vi "TestGit01.vi"() -> ()   [LabVIEW 2025]
uses:
  <vilib>/Analysis/NI_AALPro.lvlib
panel:
  in  "stop":bool
  out "Waveform Chart":dbl[](graph)
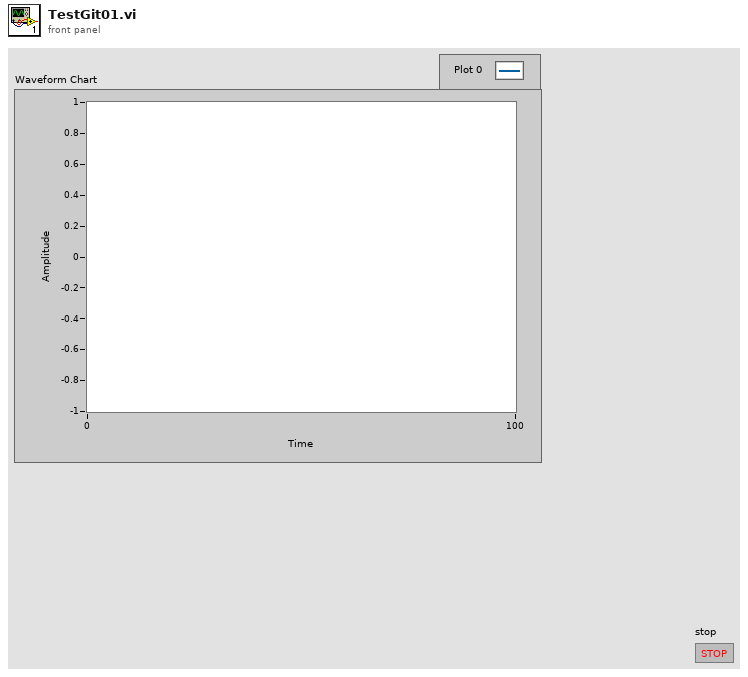
[diagram p1: front panel]
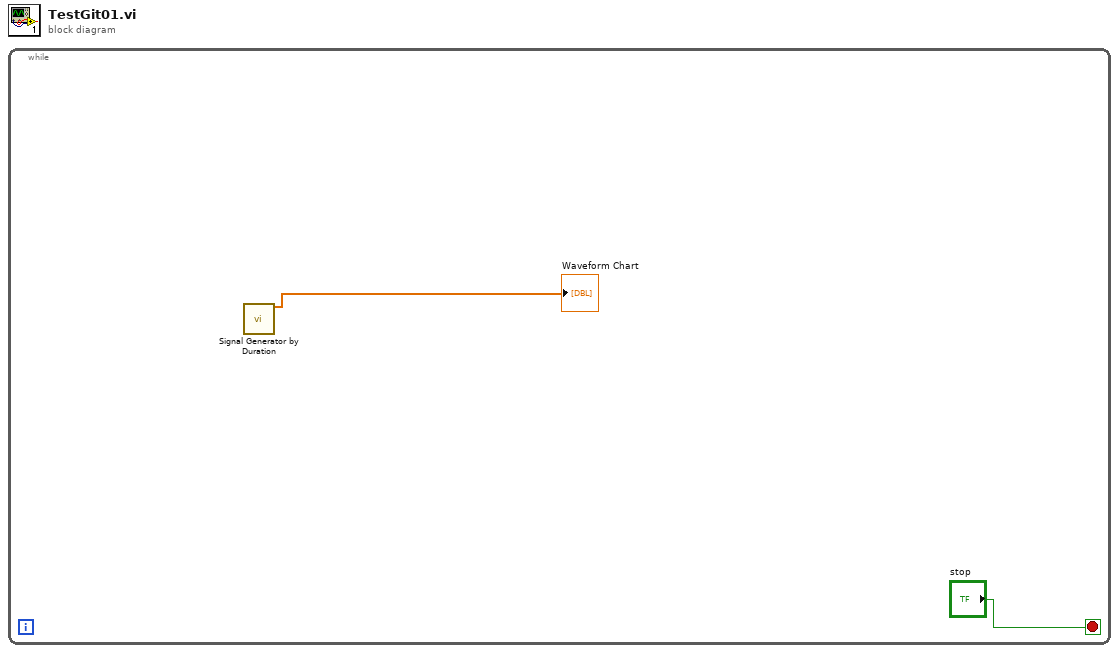
[diagram p0: block diagram]
diagram:
  n1 = while {
    stop <- "stop" stop-if-true
    n2 = call <vilib>:"Signal Generator by Duration.vi"() -> ("signal"=→"Waveform Chart":dbl[])  [unwired: 12 in, 3 out]
  }
